vi "BSM Burst table nosave_formation.vi"(6 "SN [ratio]":T1, 7 "Ex info":T3, 8 "error in":errorcluster caption="エラー入力", 11 "Table CP":T2) -> (0 "error out":errorcluster caption="エラー出力", 2 "Table Tag":T4, 3 "Table CV":T5)   [LabVIEW 2018]
panel:
  out "SN":string[](array[string])
  out "Mx Intensity level [pA]":dbl
  out "BL Level [pA]":dbl
  out "Signal Intensity [pA]":dbl
  out "S/N ratio":dbl
  out "Signal Tag":string[](array[string])
  out "Time Profile A Table":string[][](table) caption="Time A Table"
  out "CP Profile A Table":string[][](table) caption="CP A Table"
  out "Signal Profile A Table":string[][](table) caption="S Table"
  out "サブセット削除後の配列":string[](array[string])
  out "Level Composition":string[](array[string])
  out "Base Ex info array":string[](array[string])
  out "Time Profile Table P":string[][](table) caption="Time Table"
  out "CP Profile Table":string[][](table) caption="CP Table"
  out "Signal Profile Table P":string[][](table) caption="S Table"
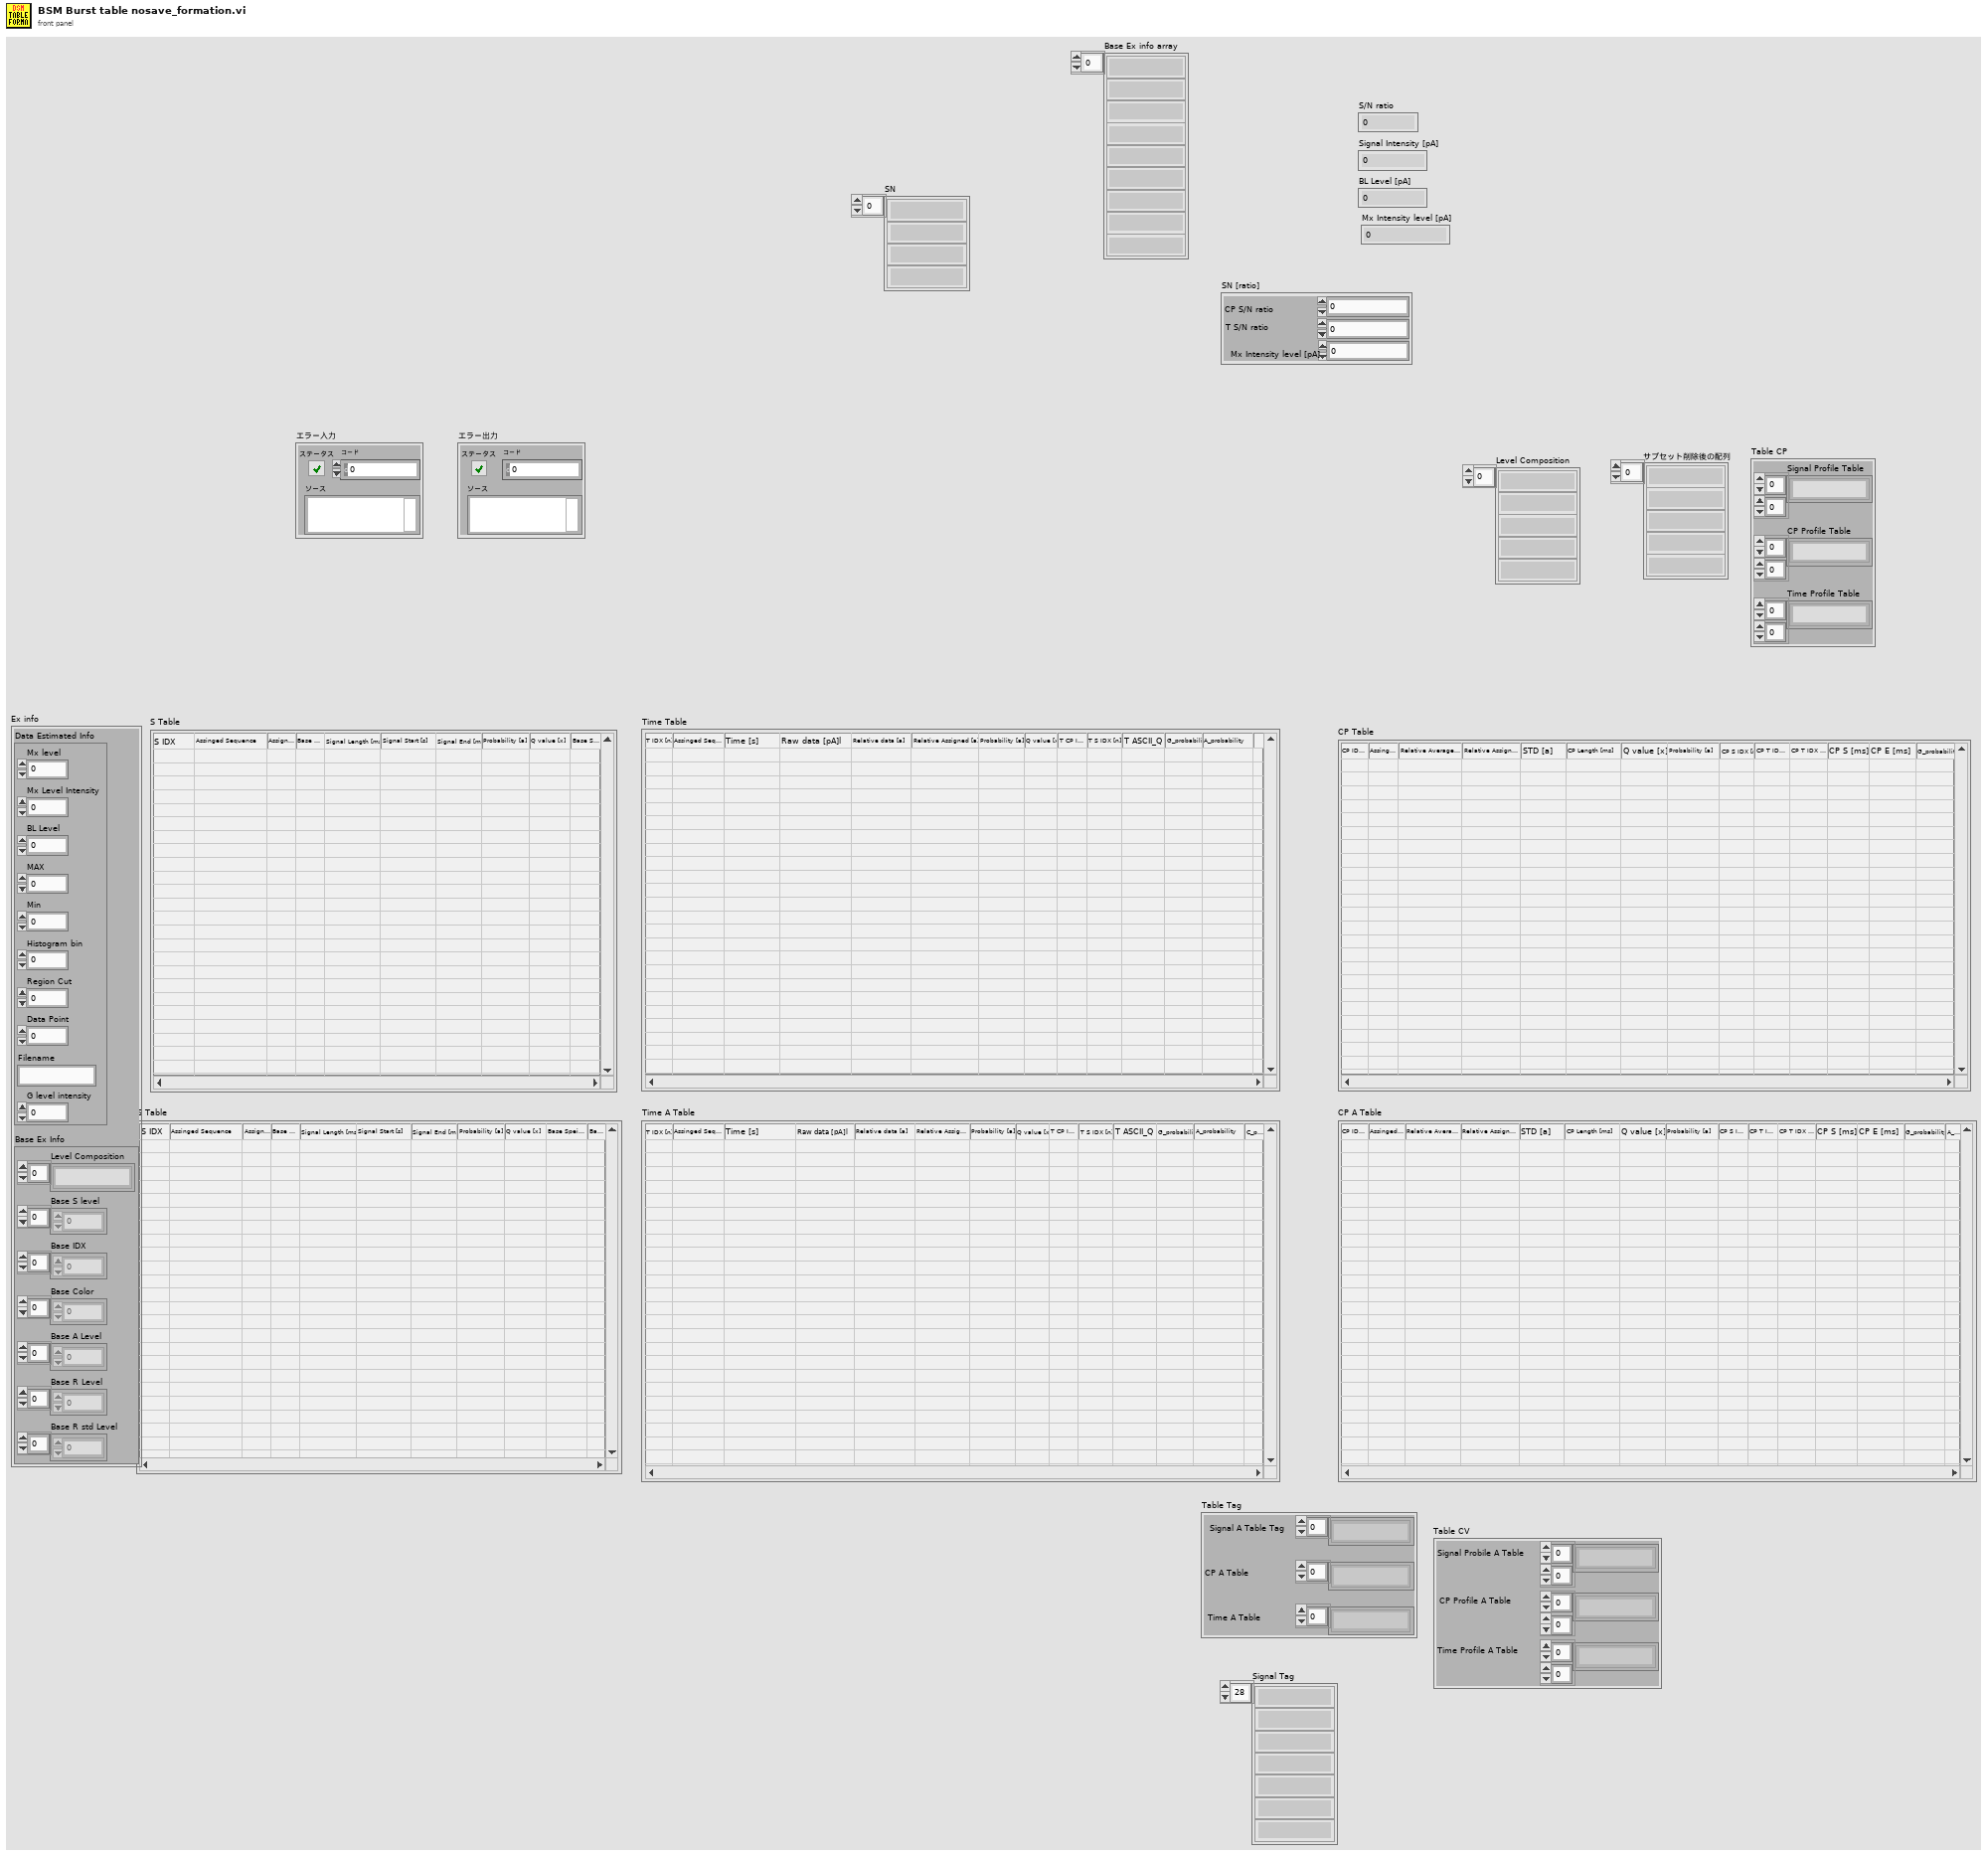
[diagram p1: front panel]
types:
  T1 = cluster{"CP S/N ratio":dbl, "T S/N ratio":dbl, "Mx Intensity level [pA]":dbl}
  T2 = cluster{"Signal Profile Table":string[][], "CP Profile Table":string[][], "Time Profile Table":string[][]}
  T3 = cluster{"Data Estimated Info":cluster{"Mx level":dbl, "Mx Level Intensity":dbl, "BL Level":dbl, "MAX":dbl, "Min":dbl, "Histogram bin":dbl, "Region Cut":dbl, "Data Point":i32, "Filename":string, "G level intensity":dbl}, "Base Ex Info":cluster{"Level Composition":string[], "Base S level":dbl[], "Base IDX":i32[], "Base Color":u32[], "Base A Level":dbl[], "Base R Level":dbl[], "Base R std Level":dbl[]}}
  T4 = cluster{"Signal A Table Tag":string[], "CP A Table":string[], "Time A Table":string[]}
  T5 = cluster{"Signal Probile A Table":string[][], "CP Profile A Table":string[][], "Time Profile A Table":string[][]}
  T6 = cluster{"Mx level":dbl, "Mx Level Intensity":dbl, "BL Level":dbl, "MAX":dbl, "Min":dbl, "Histogram bin":dbl, "Region Cut":dbl, "Data Point":i32, "Filename":string, "G level intensity":dbl}
  T7 = cluster{"Level Composition":string[], "Base S level":dbl[], "Base IDX":i32[], "Base Color":u32[], "Base A Level":dbl[], "Base R Level":dbl[], "Base R std Level":dbl[]}
  T8 = cluster{"行ヘッダ文字列[]":string[], "行ヘッダ文字列[]":string[], "行ヘッダ文字列[]":string[]}
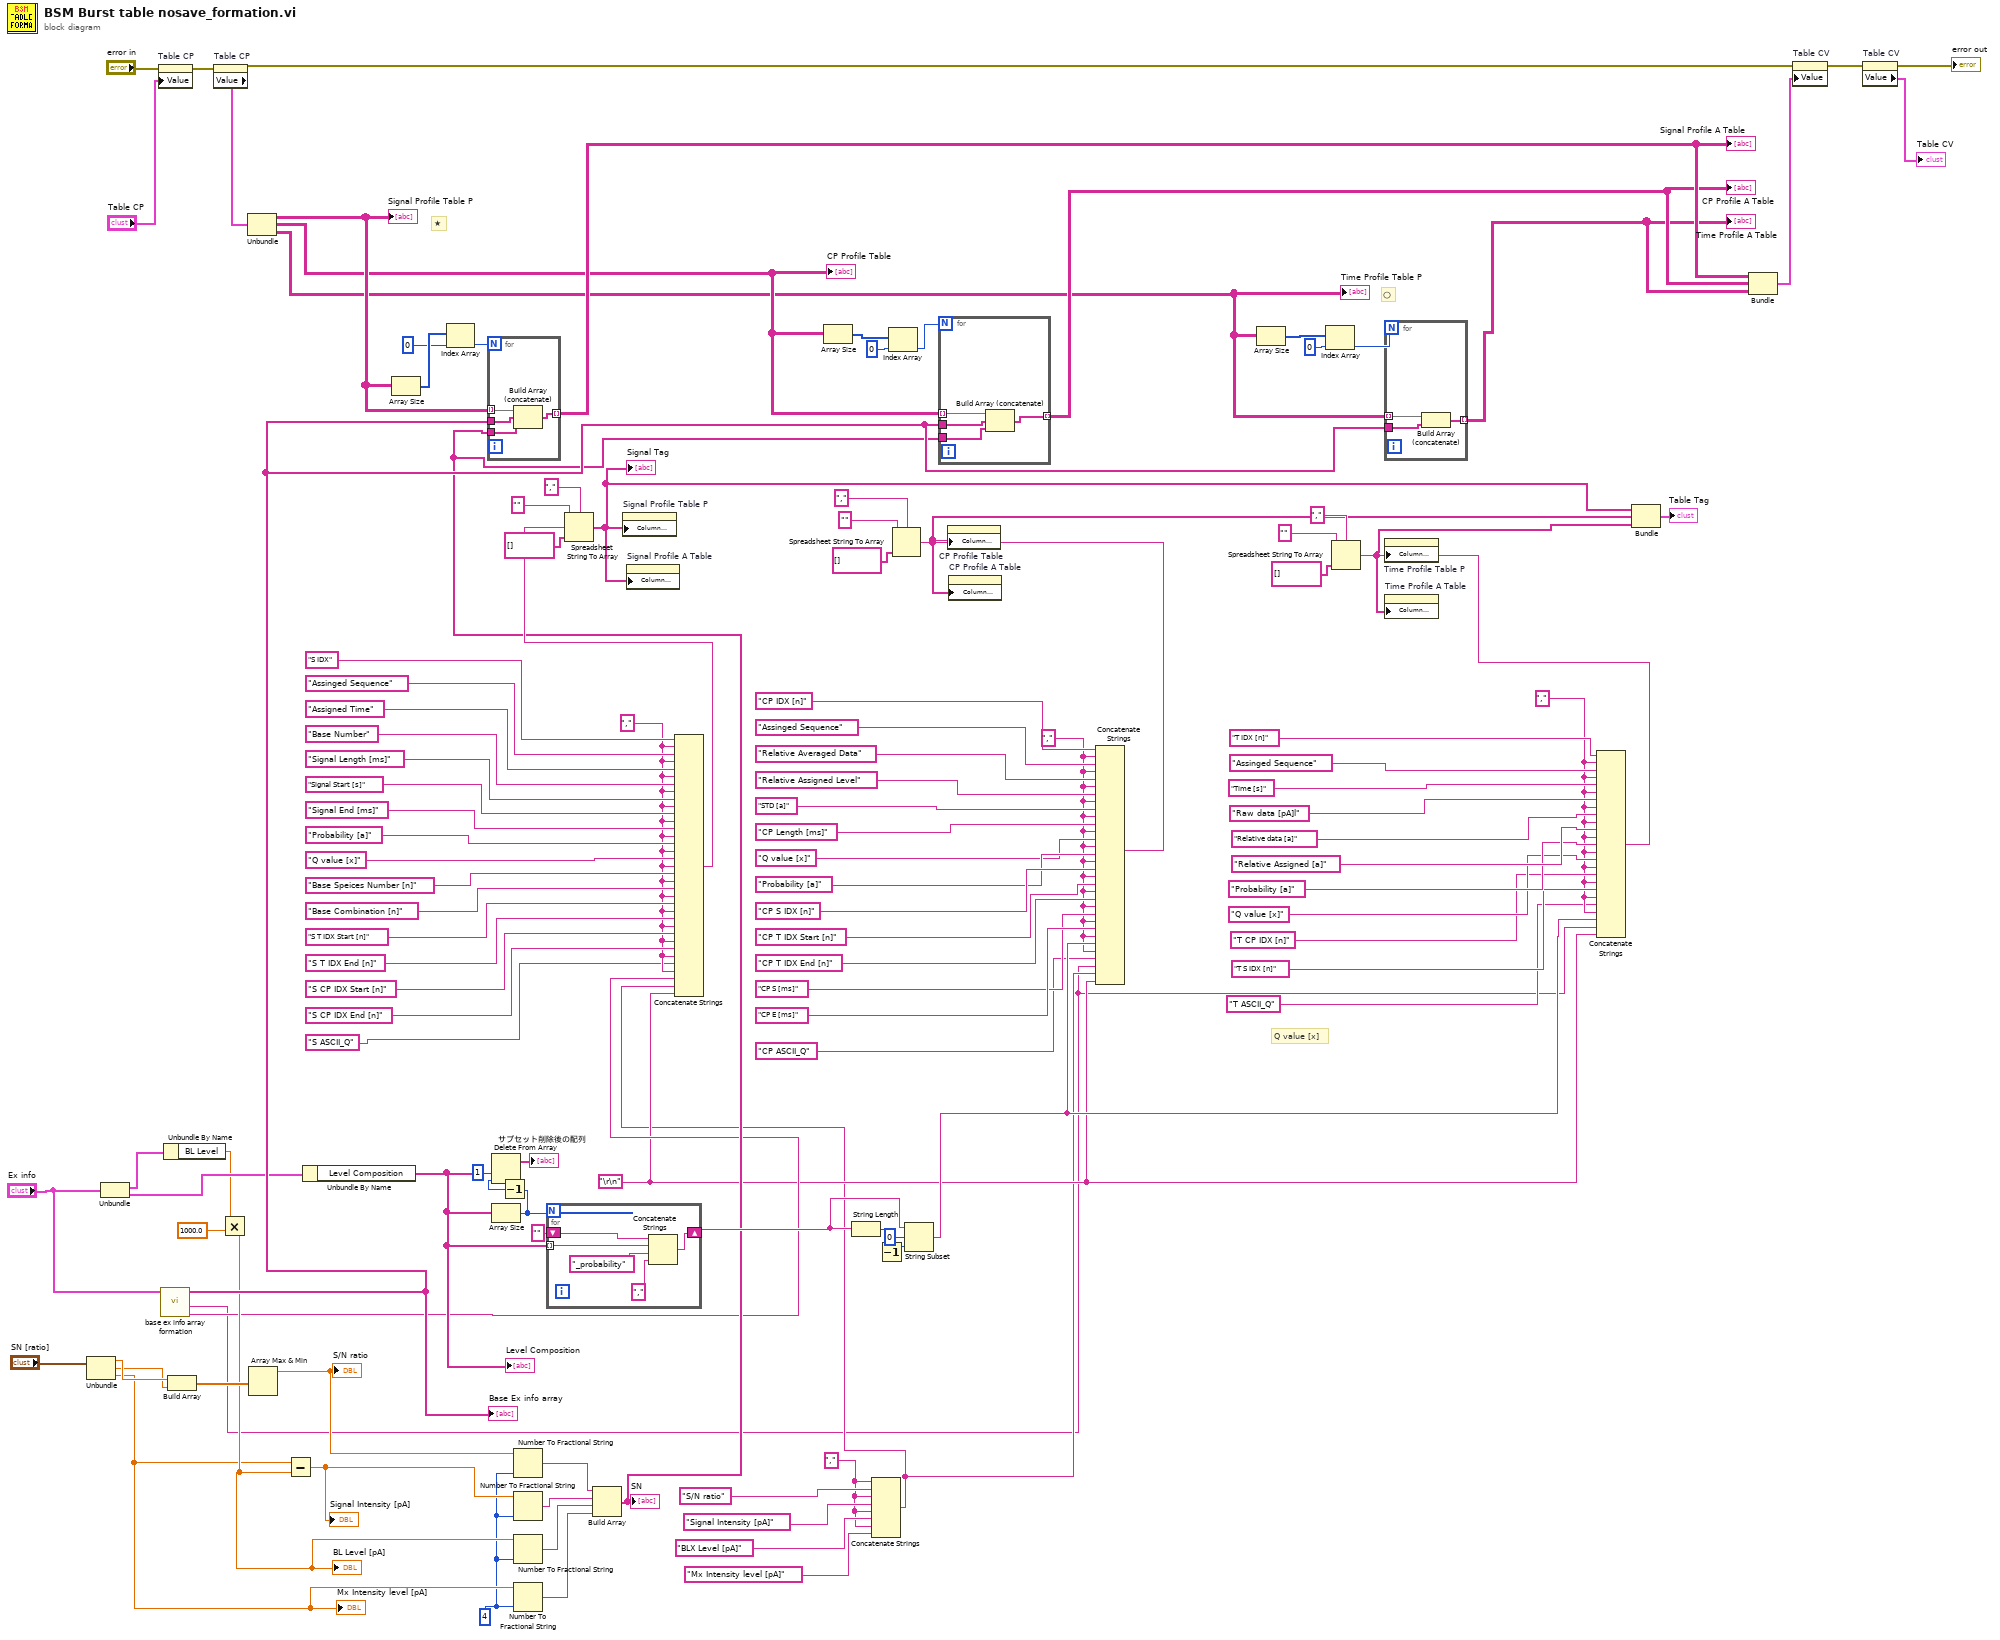
[diagram p0: block diagram]
diagram:
  w22 = "," ("デリミタ（タブ）")
  w31 = i16 4 ("精度（6）")
  w10 = "," ("デリミタ（タブ）")
  w2 = "," ("デリミタ（タブ）")
  w7 = "," ("デリミタ（タブ）")
  w5 = "\r\n"
  # "〇"
  # "★"
  # "Q value [x]"
  n1 = Unbundle("SN [ratio]") -> ("CP S/N ratio"=w40:dbl, "T S/N ratio"=w39:dbl, "Mx Intensity level [pA]"=w32:dbl)
  "Mx Intensity level [pA]" <- w32
  n2 = Unbundle("Ex info") -> ("Data Estimated Info"=w42:T6, "Base Ex Info"=w44:T7)
  n3 = property on="Table CP" class="Clust (strict)"(error in="error in", "Value"="Table CP") -> (error out=w13:errorcluster)  [unwired: 1 in, 1 out]
  n4 = call "base ex info array formation.vi"("Ex info"="Ex info") -> ("Tag"=w8:string, "Tag 2"=w3:string, "Base Ex info array"=w68:string[])  [unwired: 8 in]
  "Base Ex info array" <- w68
  n5 = Unbundle By Name(w42) -> ("BL Level"=w37:dbl)
  n6 = Build Array(w40, w39) -> (w38:dbl[])
  n7 = property on="Table CP" class="Clust (strict)"(error in=w13) -> (error out=w12:errorcluster, "Value"=w14:T2)  [unwired: 1 in, 1 out]
  n8 = Multiply(x=w37, y=1000.0) -> (x*y=w33:dbl)
  "BL Level [pA]" <- w33
  n9 = Unbundle(w14) -> ("Signal Profile Table"=w47:string[][], "CP Profile Table"=w46:string[][], "Time Profile Table"=w45:string[][])
  "Signal Profile Table P" <- w47
  "CP Profile Table" <- w46
  "Time Profile Table P" <- w45
  n10 = Array Max & Min(array=w38) -> (max value=w35:dbl)  [unwired: 3 out]
  "S/N ratio" <- w35
  n11 = Subtract(x=w32, y=w33) -> (x-y=w34:dbl)
  "Signal Intensity [pA]" <- w34
  n12 = Unbundle By Name(w44) -> ("Level Composition"=w43:string[])
  "Level Composition" <- w43
  n13 = Array Size(array=w47) -> (size(s)=w80:i32[])
  n14 = Index Array(array=w80, index=0 ("指標")) -> (element=w78:i32)
  n15 = Array Size(array=w43) -> (size(s)=w99:i32)
  n16 = Decrement(x=w99) -> (x-1=w100:i32)
  n17 = Delete From Array(array=w43, length=1 ("長さ"), index=w100) -> (array with subset deleted=→"サブセット削除後の配列":string[])  [unwired: 1 out]
  n18 = Number To Fractional String(number=w35, precision (6)=w31) -> (F-format string=w30:string)  [unwired: 2 in]
  n19 = Number To Fractional String(number=w34, precision (6)=w31) -> (F-format string=w29:string)  [unwired: 2 in]
  n20 = Number To Fractional String(number=w33, precision (6)=w31) -> (F-format string=w28:string)  [unwired: 2 in]
  n21 = Number To Fractional String(number=w32, precision (6)=w31) -> (F-format string=w27:string)  [unwired: 2 in]
  n22 = for {
    N: w99 -> [_]
    tunnel: w43 -> [w129] mode=indexing
    shift-right: [w128] -> w94
    shift-left: "" -> [w127]
    n23 = Concatenate Strings(w127, w129, "_probability" ("文字列"), "," ("デリミタ（タブ）")) -> (w128:string)
  }
  n24 = Build Array(w30, w29, w28, w27) -> (w21:string[])
  "SN" <- w21
  n25 = for {
    N: w78 -> [_]
    tunnel: w47 -> [w133] mode=indexing
    tunnel: w68 -> [w132]
    tunnel: [w131] -> w67 mode=indexing
    tunnel: w21 -> [w130]
    n26 = Build Array (concatenate)(w133, w132, w130) -> (w131:string[])
  }
  "Signal Profile A Table" <- w67
  n27 = Array Size(array=w46) -> (size(s)=w73:i32[])
  n28 = String Length(string=w94) -> (length=w96:i32)
  n29 = Concatenate Strings(w22, "S/N ratio" ("書き込みバッファ"), w22, "Signal Intensity [pA]" ("書き込みバッファ"), w22, "BLX Level [pA]" ("書き込みバッファ"), w22, "Mx Intensity level [pA]" ("書き込みバッファ")) -> (w4:string)
  n30 = Concatenate Strings("S IDX" ("文字列"), w7, "Assinged Sequence" ("書き込みバッファ"), w7, "Assigned Time" ("書き込みバッファ"), w7, "Base Number" ("書き込みバッファ"), w7, "Signal Length [ms]" ("書き込みバッファ"), w7, "Signal Start [s]" ("書き込みバッファ"), w7, "Signal End [ms]" ("書き込みバッファ"), w7, "Probability [a]" ("書き込みバッファ"), w7, "Q value [x]" ("書き込みバッファ"), w7, "Base Speices Number [n]" ("書き込みバッファ"), w7, "Base Combination [n]" ("書き込みバッファ"), w7, "S T IDX Start [n]" ("書き込みバッファ"), w7, "S T IDX End [n]" ("書き込みバッファ"), w7, "S CP IDX Start [n]" ("書き込みバッファ"), w7, "S CP IDX End [n]" ("書き込みバッファ"), w7, "S ASCII_Q" ("書き込みバッファ"), w7, w8, w4, w5) -> (w90:string)
  n31 = Spreadsheet String To Array(delimiter (Tab)="," ("デリミタ（タブ）"), format string="" ("形式文字列"), spreadsheet string=w90, array type (2D Dbl)=string[] [] ("行ヘッダ文字列[]")) -> (array=w64:string[])
  "Signal Tag" <- w64
  n32 = property on="Signal Profile Table P" class="Tbl (strict)"("Column Headers[]"=w64) -> ()  [unwired: 2 in, 2 out]
  n33 = property on="Signal Profile A Table" class="Tbl (strict)"("Column Headers[]"=w64) -> ()  [unwired: 2 in, 2 out]
  n34 = Decrement(x=w96) -> (x-1=w95:i32)
  n35 = Index Array(array=w73, index=0 ("指標")) -> (element=w71:i32)
  n36 = String Subset(string=w94, offset (0)=0 ("オフセット（0）"), length (rest)=w95) -> (substring=w11:string)
  n37 = for {
    N: w71 -> [_]
    tunnel: w46 -> [w137] mode=indexing
    tunnel: w68 -> [w136]
    tunnel: [w135] -> w66 mode=indexing
    tunnel: w21 -> [w134]
    n38 = Build Array (concatenate)(w137, w136, w134) -> (w135:string[])
  }
  "CP Profile A Table" <- w66
  n39 = Concatenate Strings("CP IDX [n]" ("文字列"), w2, "Assinged Sequence" ("書き込みバッファ"), w2, "Relative Averaged Data" ("書き込みバッファ"), w2, "Relative Assigned Level" ("書き込みバッファ"), w2, "STD [a]" ("書き込みバッファ"), w2, "CP Length [ms]" ("書き込みバッファ"), w2, "Q value [x]" ("書き込みバッファ"), w2, "Probability [a]" ("書き込みバッファ"), w2, "CP S IDX [n]" ("書き込みバッファ"), w2, "CP T IDX Start [n]" ("書き込みバッファ"), w2, "CP T IDX End [n]" ("書き込みバッファ"), w2, "CP S [ms]" ("書き込みバッファ"), w2, "CP E [ms]" ("書き込みバッファ"), w2, w11, w2, "CP ASCII_Q" ("書き込みバッファ"), w3, w4, w5) -> (w83:string)
  n40 = Spreadsheet String To Array(delimiter (Tab)="," ("デリミタ（タブ）"), format string="" ("形式文字列"), spreadsheet string=w83, array type (2D Dbl)=string[] [] ("行ヘッダ文字列[]")) -> (array=w63:string[])
  n41 = property on="CP Profile Table" class="Tbl (strict)"("Column Headers[]"=w63) -> ()  [unwired: 2 in, 2 out]
  n42 = property on="CP Profile A Table" class="Tbl (strict)"("Column Headers[]"=w63) -> ()  [unwired: 2 in, 2 out]
  n43 = Array Size(array=w45) -> (size(s)=w70:i32[])
  n44 = Index Array(array=w70, index=0 ("指標")) -> (element=w48:i32)
  n45 = for {
    N: w48 -> [_]
    tunnel: w45 -> [w140] mode=indexing
    tunnel: w68 -> [w139]
    tunnel: [w138] -> w65 mode=indexing
    n46 = Build Array (concatenate)(w140, w139) -> (w138:string[])
  }
  "Time Profile A Table" <- w65
  n47 = Concatenate Strings("T IDX [n]" ("文字列"), w10, "Assinged Sequence" ("書き込みバッファ"), w10, "Time [s]" ("書き込みバッファ"), w10, "Raw data [pA]l" ("書き込みバッファ"), w10, "Relative data [a]" ("書き込みバッファ"), w10, "Relative Assigned [a]" ("書き込みバッファ"), w10, "Probability [a]" ("書き込みバッファ"), w10, "Q value [x]" ("書き込みバッファ"), w10, "T CP IDX [n]" ("書き込みバッファ"), w10, "T S IDX [n]" ("書き込みバッファ"), w10, "T ASCII_Q" ("書き込みバッファ"), w10, w11, w3, w5) -> (w82:string)
  n48 = Spreadsheet String To Array(delimiter (Tab)="," ("デリミタ（タブ）"), format string="" ("形式文字列"), spreadsheet string=w82, array type (2D Dbl)=string[] [] ("行ヘッダ文字列[]")) -> (array=w62:string[])
  n49 = property on="Time Profile Table P" class="Tbl (strict)"("Column Headers[]"=w62) -> ()  [unwired: 2 in, 2 out]
  n50 = property on="Time Profile A Table" class="Tbl (strict)"("Column Headers[]"=w62) -> ()  [unwired: 2 in, 2 out]
  n51 = Bundle("行ヘッダ文字列[]"=w64, "行ヘッダ文字列[]"=w63, "行ヘッダ文字列[]"=w62) -> (→"Table Tag":T8)  [unwired: 1 in]
  n52 = Bundle(w67, w66, w65) -> (w20:cluster{string[][], string[][], string[][]})  [unwired: 1 in]
  n53 = property on="Table CV" class="Clust (strict)"(error in=w12, "Value"=w20) -> (error out=w18:errorcluster)  [unwired: 1 in, 1 out]
  n54 = property on="Table CV" class="Clust (strict)"(error in=w18) -> (error out=→"error out":errorcluster, "Value"=→"Table CV":T5)  [unwired: 1 in, 1 out]
